vi "Create.vi"(5 "OpenMetrics Compliant?":bool=TRUE, 6 "Label Names":string[](array[string]), 7 "Registry Name":string="_default_registry", 8 "error in (no error)":errorcluster, 9 "Auto-register?":bool=TRUE, 10 "Description":string, 11 "Metric Name":string) -> (0 "error out":errorcluster, 3 "Counter Ref":refnum<data-value>)   [LabVIEW 2020, in "Metrics.lvlib" / "Counter.lvclass"]
doc: "Creates a new Counter metric. A counter is a metric that can only go up (by one, or more)."
uses:
  Counter.lvclass
  C:/Github-locals/PromVIEW/src/metrics/metric/Metric.lvclass
  metric/Metric.lvclass/Metric.ctl
  metric/Write Name.vi
  metric/Write Description.vi
  metric/Write Label Names.vi
  metric/Validate Name.vi
  registry/session/Registry Session.lvclass
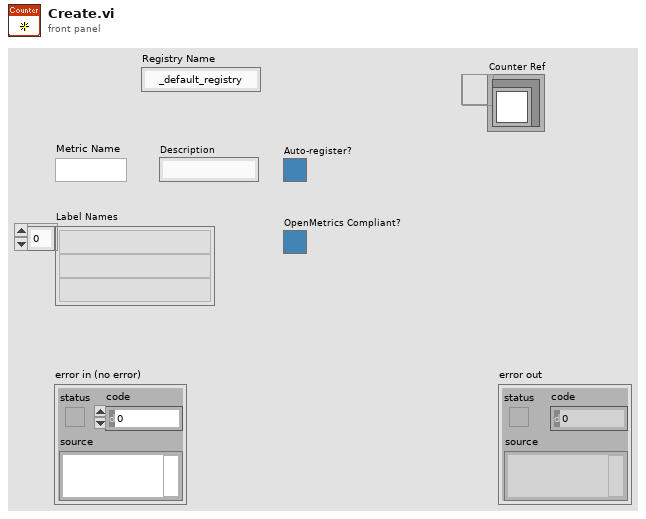
[diagram p1: front panel]
types:
  T1 = typedef "Registry.lvlib/Registry Session.lvclass/Session Handle.ctl" = refnum<data-value>
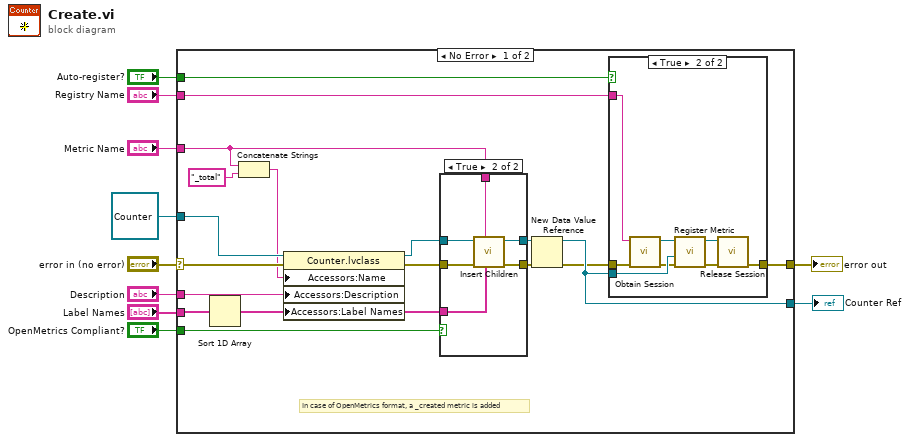
[diagram p0: block diagram]
diagram:
  n1 = case shown="No Error" "error in (no error)" {
    selector: "error in (no error)" -> [w18 w46]
    tunnel: [w23 w46] -> w9
    tunnel: "Metric Name" -> [w22 _]
    tunnel: "Label Names" -> [w12 _]
    tunnel: "Description" -> [w26 _]
    tunnel: refnum<class "Counter.lvclass"> refnum ("Metrics.lvlib:Counter.lvclass") -> [w27 _]
    tunnel: [w21 _] -> w4
    tunnel: "Registry Name" -> [w24 _]
    tunnel: "Auto-register?" -> [w19 _]
    tunnel: "OpenMetrics Compliant?" -> [w16 _]
    frame No Error {
      # "In case of OpenMetrics format, a _created metric is added"
      n2 = Sort 1D Array(array=w12) -> (sorted array=w11:string[])
      n3 = Concatenate Strings(w22, "_total" ("string")) -> (w13:string)
      n4 = property class="Counter.lvclass"(reference=w27, error in=w18, "Accessors:Name"=w13, "Accessors:Description"=w26, "Accessors:Label Names"=w11) -> (reference out=w25:refnum<class "Counter.lvclass">, error out=w17:errorcluster)
      n5 = case shown="True" w16 {
        tunnel: w25 -> [w30 w36]
        tunnel: w17 -> [w29 w35]
        tunnel: w22 -> [_ w32]
        tunnel: [w29 w34] -> w15
        tunnel: [w30 w33] -> w14
        tunnel: w11 -> [_ w31]
        frame False {
        }
        frame True {
          n6 = call "Insert Children.vi"("Label Names"=w31, "Metric Name"=w32, "error in (no error)"=w35, "Counter in"=w36) -> ("error out"=w34:errorcluster, "Counter out"=w33:refnum<class "Counter.lvclass">)  [unwired: 6 in]
        }
      }
      n7 = New Data Value Reference(data value=w14, error in=w15) -> (data value reference=w21:refnum<data-value>, error out=w20:errorcluster)
      n8 = case shown="True" w19 {
        tunnel: w24 -> [_ w45]
        tunnel: [w37 w39] -> w23
        tunnel: w21 -> [_ w44]
        tunnel: w20 -> [w37 w42]
        frame False {
        }
        frame True {
          n9 = call "Obtain Session.vi"("error in (no error)"=w42, "Session  Name ()"=w45) -> ("error out"=w41:errorcluster, "Session Handle"=w43:T1)  [unwired: 8 in]
          n10 = call "Register Metric.vi"("error in (no error)"=w41, "New Metric"=w44, "Session Handle in"=w43) -> ("error out"=w40:errorcluster, "Session Handle out"=w38:T1)  [unwired: 7 in]
          n11 = call "Release Session.vi"("error in (no error)"=w40, "Session Handle"=w38) -> ("error out"=w39:errorcluster)  [unwired: 9 in]
        }
      }
    }
    frame Error {
    }
  }
  "error out" <- w9
  "Counter Ref" <- w4
